vi "packet_receive.vi"(11 "버퍼 in":string) -> (0 "D1":u8, 1 "CMD":u8, 2 "유효":bool, 3 "버퍼 out":string, 4 "D2":u8)   [LabVIEW 2026]
panel:
  out "패킷 다 옴":bool
  out "STX 위치":i32
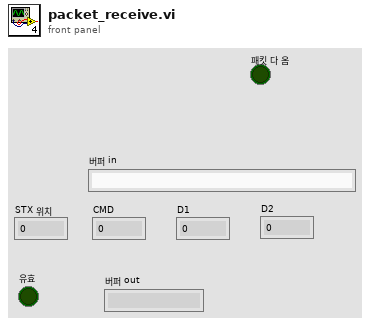
[diagram p1: front panel]
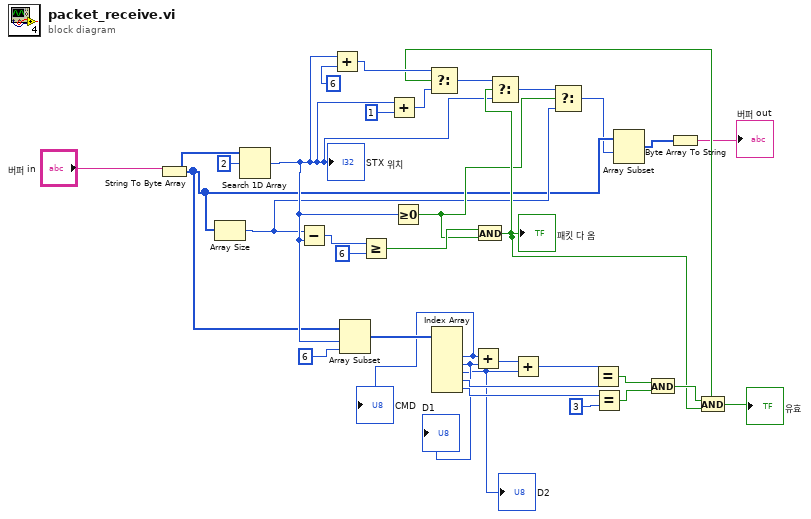
[diagram p0: block diagram]
diagram:
  n1 = String To Byte Array(string="버퍼 in") -> (unsigned byte array=w4:u8[])
  n2 = Array Size(array=w4) -> (size(s)=w5:i32)
  n3 = Search 1D Array(1D array=w4, element=u8 2) -> (index of element=w8:i32)  [unwired: 1 in]
  "STX 위치" <- w8
  n4 = Subtract(x=w5, y=w8) -> (x-y=w31:i32)
  n5 = Add(x=w8, y=6) -> (x+y=w13:i32)
  n6 = Array Subset(array=w4, index=w8, length=6) -> (w27:u8[])
  n7 = Greater Or Equal?(x=w31, y=6) -> (x >= y?=w29:bool)
  n8 = Add(x=w8, y=1) -> (x+y=w12:i32)
  n9 = Greater Or Equal To 0?(x=w8) -> (x >= 0?=w6:bool)
  n10 = Index Array(array=w27) -> (element #2=w18:u8, element #3=w17:u8, element #4=w16:u8, element #5=w24:u8, element #6=w23:u8)  [unwired: 6 in, 1 out]
  "CMD" <- w18
  "D1" <- w17
  "D2" <- w16
  n11 = Add(x=w18, y=w17) -> (x+y=w26:u8)
  n12 = And(x=w29, y=w6) -> (x .and. y?=w9:bool)
  "패킷 다 옴" <- w9
  n13 = Add(x=w26, y=w16) -> (x+y=w25:u8)
  n14 = Equal?(x=w24, y=w25) -> (x = y?=w21:bool)
  n15 = Equal?(x=w23, y=u8 3) -> (x = y?=w20:bool)
  n16 = And(x=w21, y=w20) -> (x .and. y?=w19:bool)
  n17 = And(x=w19, y=w9) -> (x .and. y?=w11:bool)
  "유효" <- w11
  n18 = Select(t=w13, s=w11, f=w12) -> (s? t:f=w10:i32)
  n19 = Select(t=w10, s=w9, f=w8) -> (s? t:f=w7:i32)
  n20 = Select(t=w7, s=w6, f=w5) -> (s? t:f=w3:i32)
  n21 = Array Subset(array=w4, index=w3) -> (w2:u8[])  [unwired: 1 in]
  n22 = Byte Array To String(unsigned byte array=w2) -> (string=→"버퍼 out":string)
